vi "set Marker All Off.vi"(8 "error in (no error)":errorcluster, 11 "FSV-40N in":refnum<class "FSV-40N.lvclass">) -> (0 "error out":errorcluster, 3 "FSV-40N out":refnum<class "FSV-40N.lvclass">)   [LabVIEW 2023, in "Spectrum Analyzer.lvlib" / "FSV-40N.lvclass"]
uses:
  FSV-40N.lvclass
  FSV-40N.lvclass/FSV-40N.ctl
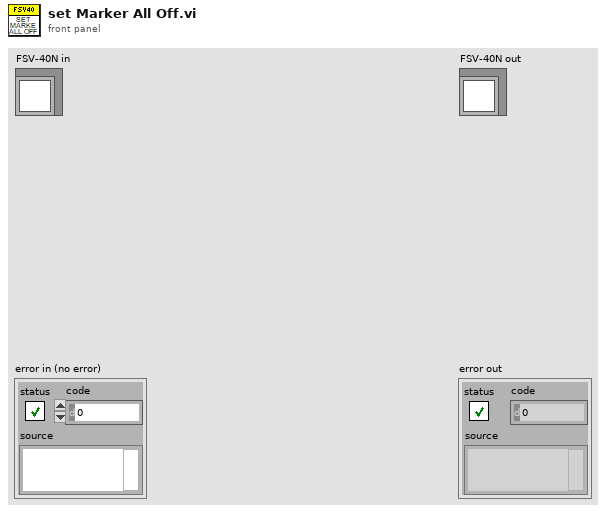
[diagram p1: front panel]
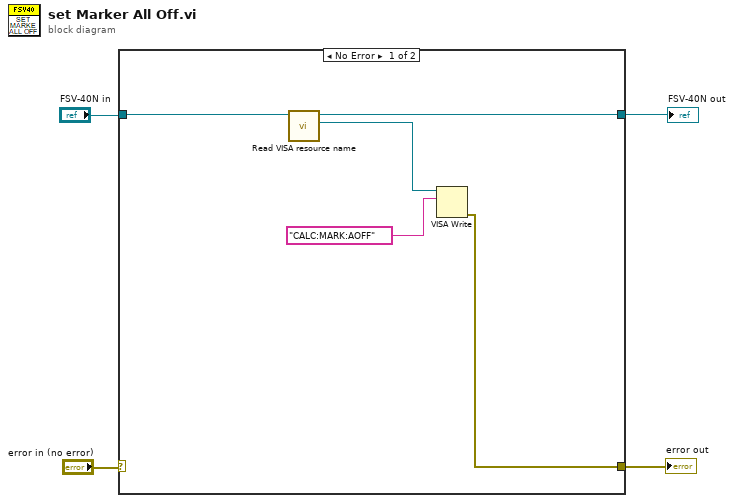
[diagram p0: block diagram]
diagram:
  n1 = case shown="No Error" "error in (no error)" {
    selector: "error in (no error)" -> [_ w10]
    tunnel: "FSV-40N in" -> [w9 w11]
    tunnel: [w6 w11] -> w4
    tunnel: [w8 w10] -> w2
    frame No Error {
      n2 = call "Read VISA resource name.vi"("FSV-40N in"=w9) -> ("VISA resource name"=w7:refnum<visa-resource-name>, "FSV-40N out"=w6:refnum<class "FSV-40N.lvclass">)  [unwired: 8 in, 1 out]
      n3 = VISA Write(VISA resource name=w7, write buffer="CALC:MARK:AOFF") -> (error out=w8:errorcluster)  [unwired: 1 in, 2 out]
    }
    frame Error {
    }
  }
  "error out" <- w2
  "FSV-40N out" <- w4
